vi "_Buffer_To_AllElements.vi"(10 "count (-1: all)":i32=-1, 11 "Buffer":refnum<class "VariantBuffer.lvclass">) -> (3 "elements":variant[](array[variant]))   [LabVIEW 2013, in "CircularBuffer.lvlib" / "VariantBuffer.lvclass"]
uses:
  VariantBuffer.lvclass
  VariantBuffer.lvclass/VariantBuffer.ctl
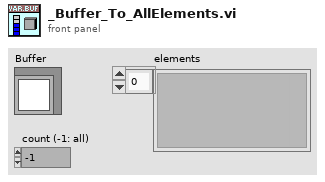
[diagram p1: front panel]
types:
  T1 = typedef "CircularBuffer.lvlib/VariantBuffer.lvclass/buffer-type -- enum.ctl" = enum16{"Queue", "Stack"}
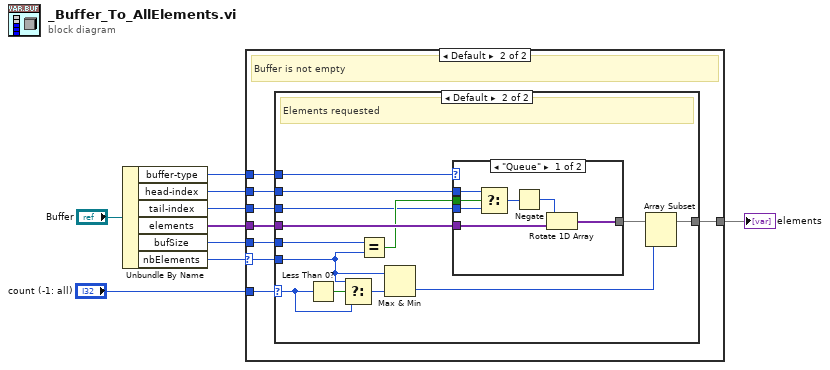
[diagram p0: block diagram]
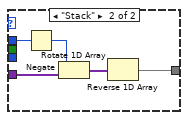
[diagram p4: hidden frame]
diagram:
  n1 = Unbundle By Name("Buffer") -> ("buffer-type"=w2:T1, "head-index"=w3:i32, "tail-index"=w9:i32, "elements"=w6:variant[], "bufSize"=w5:i32, "nbElements"=w1:i32)
  n2 = case shown="Default" w1 {
    selector: w1 -> [_ w13]
    tunnel: "count (-1: all)" -> [_ w12]
    tunnel: w9 -> [_ w17]
    tunnel: [_ w16] -> w8
    tunnel: w6 -> [_ w15]
    tunnel: w5 -> [_ w14]
    tunnel: w2 -> [_ w11]
    tunnel: w3 -> [_ w10]
    frame 0 {
      # "Buffer is empty"
    }
    frame Default {
      # "Buffer is not empty"
      n3 = case shown="Default" w12 {
        selector: w12 -> [_ w26]
        tunnel: w17 -> [_ w22]
        tunnel: [_ w28] -> w16
        tunnel: w15 -> [_ w27]
        tunnel: w14 -> [_ w25]
        tunnel: w13 -> [_ w19]
        tunnel: w11 -> [_ w18]
        tunnel: w10 -> [_ w23]
        frame 0 {
          # "No elements are requested"
        }
        frame Default {
          # "Elements requested"
          n4 = Less Than 0?(x=w26) -> (x < 0?=w29:bool)
          n5 = Select(t=w19, s=w29, f=w26) -> (s? t:f=w30:i32)
          n6 = Equal?(x=w25, y=w19) -> (x = y?=w24:bool)
          n7 = Max & Min(x=w19, y=w30) -> (min(x,y)=w21:i32)  [unwired: 1 out]
          n8 = case shown="\"Queue\"" w18 {
            tunnel: w27 -> [w37 w42]
            tunnel: w24 -> [w36 _]
            tunnel: w23 -> [w35 w38]
            tunnel: w22 -> [w34 _]
            tunnel: [w31 w39] -> w20
            frame "Queue" {
              n9 = Select(t=w35, s=w36, f=w34) -> (s? t:f=w33:i32)
              n10 = Negate(x=w33) -> (-x=w32:i32)
              n11 = Rotate 1D Array(1:w37, 2:w32) -> (0:w31:variant[])
            }
            frame "Stack" {
              n12 = Negate(x=w38) -> (-x=w41:i32)
              n13 = Rotate 1D Array(1:w42, 2:w41) -> (0:w40:variant[])
              n14 = Reverse 1D Array(array=w40) -> (reversed array=w39:variant[])
            }
          }
          n15 = Array Subset(array=w20, length=w21) -> (w28:variant[])  [unwired: 1 in]
        }
      }
    }
  }
  "elements" <- w8
